vi "KalmanFilter_Predict.vi"(6 "dT_Seconds":dbl=0.02, 10 "U":T2, 11 "in KalmanFilter":T1) -> (0 "Error":bool, 3 "out KalmanFilter":T1)   [LabVIEW 2019, in "Trajectory_Library.lvlib"]
doc: "Project the model into the future with a new control input u.\n \nInputs:\n - inKalmanFilter -- filter data cluster\n - u -- New control input from controller.\n - dtSeconds -- Timestep for prediction. \n\nOutputs:\n - outKalmanFilter -- updated filter data cluster\n - error -- If value is TRUE, an error occured."
uses:
  Trajectory_Library.lvlib
  <vilib>/Analysis/Matrix/Datatypes/RealMatrix.ctl
  <vilib>/Analysis/Matrix/NI_Matrix.lvlib
  TypeDef/LINEAR_SYSTEM.ctl
  TypeDef/KALMAN_FILTER.ctl
panel:
  # "<Inputs,1>"
  # "Steady State Gain  \n<States,Outputs>"
  # "State Estimate <Statess,1>"
  # "<States,States>"
  # "<States,Inputs>"
  # "<Outputs,States>"
  # "<Outputs,Inputs>"
  # "Steady State Gain  \n<States,Outputs>"
  # "State Estimate <Statess,1>"
  # "<States,States>"
  # "<States,Inputs>"
  # "<Outputs,States>"
  # "<Outputs,Inputs>"
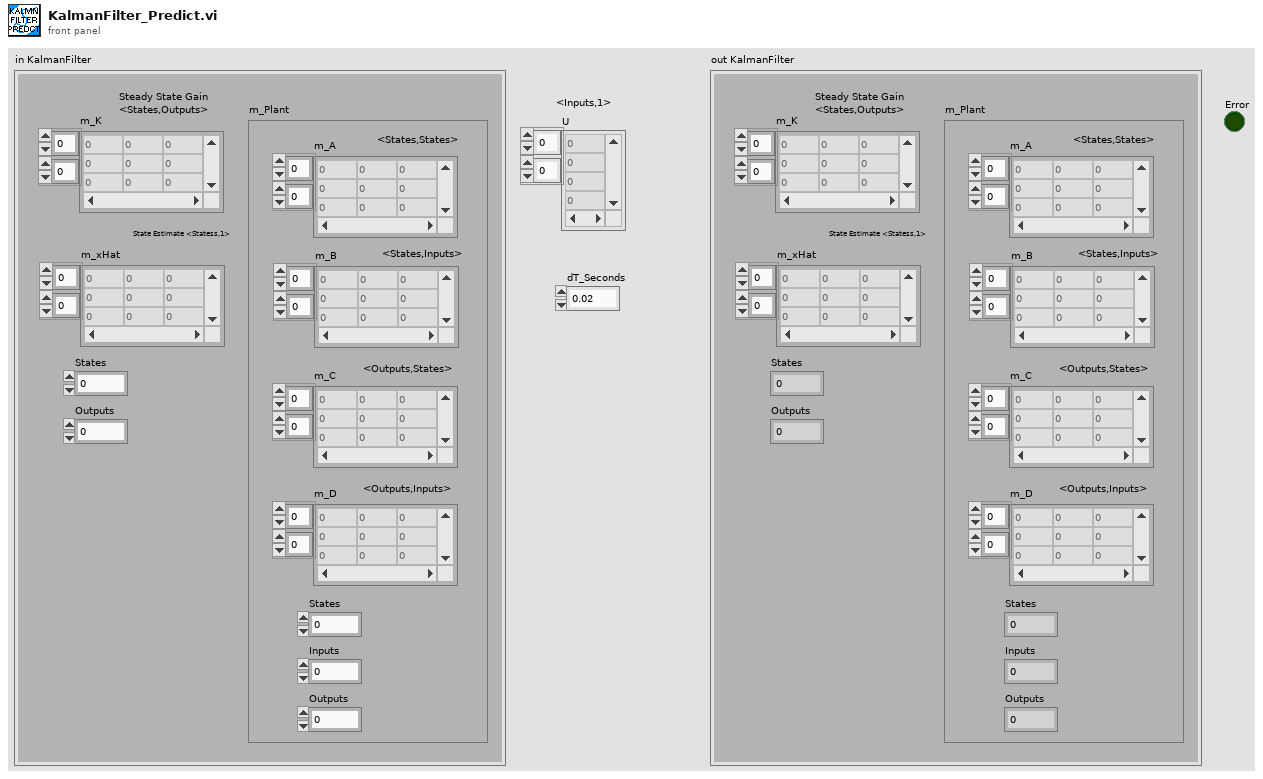
[diagram p1: front panel]
types:
  T1 = typedef "Trajectory_Library.lvlib/KALMAN_FILTER.ctl" = cluster{"m_K":T2, "m_xHat":T2, "States":i32, "Outputs":i32, "m_Plant":T3}
  T2 = typedef "NI_Matrix.lvlib/RealMatrix.ctl" = dbl[][]
  T3 = typedef "Trajectory_Library.lvlib/LINEAR_SYSTEM.ctl" = cluster{"m_A":T2, "m_B":T2, "m_C":T2, "m_D":T2, "States":i32, "Inputs":i32, "Outputs":i32}
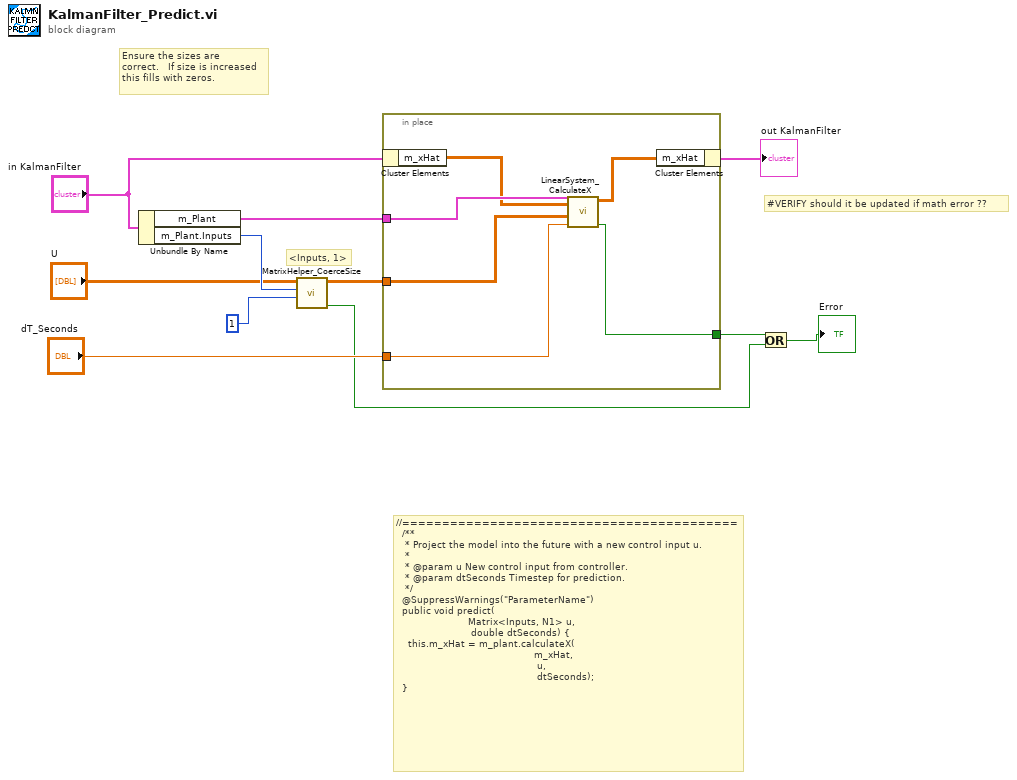
[diagram p0: block diagram]
diagram:
  # "//==========================================\n  /**\n   * Project the model into the future with a new control input u.\n   *\n   * @param u New control input from controller.\n   * @param dtSeconds Timestep for prediction.\n   */\n  @SuppressWarnings(\"ParameterName\")\n  public void predict(\n                        Matrix<Inputs, N1> u, \n                         double dtSeconds) {\n    this.m_xHat = m_plant.calculateX(\n                                              m_xHat, \n                                               u, \n                                               dtSeconds);\n  }"
  # "#VERIFY should it be updated if math error ??"
  # "<Inputs, 1>"
  # "Ensure the sizes are\ncorrect.   If size is increased \nthis fills with zeros."
  n1 = Unbundle By Name("in KalmanFilter") -> ("m_Plant"=w9:T3, "m_Plant.Inputs"=w7:i32)
  n2 = call "MatrixHelper_CoerceSize.vi"("Columns"=1 ("y"), "Rows"=w7, "input matrix"="U") -> ("Coerced"=w1:bool, "output matrix"=w4:T2)  [unwired: 7 in]
  n3 = in-place {
    in-place-border: w4 -> [w13]
    in-place-border: w9 -> [w17]
    in-place-border: "dT_Seconds" -> [w16]
    in-place-border: [w12] -> w3
    n4 = in-place-cluster #1("in KalmanFilter") -> ("m_xHat"=w15:T2)
    n5 = call "LinearSystem_CalculateX.vi"("dT_Seconds"=w16, "ClampedU"=w13, "X"=w15, "Linearsystem"=w17) -> ("Error"=w12:bool, "outX"=w14:T2)  [unwired: 6 in]
    n6 = in-place-cluster #1("m_xHat"=w14) -> (→"out KalmanFilter":T1)
  }
  n7 = Or(x=w3, y=w1) -> (x .or. y?=→"Error":bool)
